vi "Obtain Request Events.vi"(8 "error in":errorcluster, 10 "Create New? (F)":bool) -> (0 "error out":errorcluster, 2 "testCoordinator Request Events":T1)   [LabVIEW 2026, in "testCoordinator.lvlib"]
doc: "This VI Obtains/Creates the Requests events that will be used for other modules to communicate with the module that owns this VI. These Requests events will be accessed only via Public API methods for this module.\n\n<b>NOTE</b>: The contents of this VI are automatically generated and modified by the <b>Tools > DQMH Consortium > DQMH</b> utilities. Consider using those utilities instead of making your own modifications to this VI.\n_____\nBased on DQMH Dev Tools: Project Template 7.1.2.1547."
uses:
  testCoordinator.lvlib
  Request Events--cluster.ctl
  Stop Argument--cluster.ctl
  Do Something Argument--cluster.ctl
  Do Something Else Argument--cluster.ctl
  Do Something Else and Wait for Reply Argument--cluster.ctl
  Do Something Else and Wait (Reply Payload)--cluster.ctl
  Show Panel Argument--cluster.ctl
  Hide Panel Argument--cluster.ctl
  Get Module Execution Status Argument--cluster.ctl
  Show Diagram Argument--cluster.ctl
  Set Manual Tests Folder Location Argument--cluster.ctl
  Set Manual Tests Folder Location (Reply Payload)--cluster.ctl
  Load Test Procedure Argument--cluster.ctl
  Begin Test Execution Argument--cluster.ctl
  Process Test Procedure Metadata Argument--cluster.ctl
  Instruction Completed Argument--cluster.ctl
  Process First Instruction Argument--cluster.ctl
  Load Next Test Case Argument--cluster.ctl
  Execute Launcher Argument--cluster.ctl
panel:
  # "NOTE: The contents of this VI are automatically generated and modified by the Tools > DQMH Consortium > DQMH utilities. Consider using those utilities instead of making your own modifications to this VI."
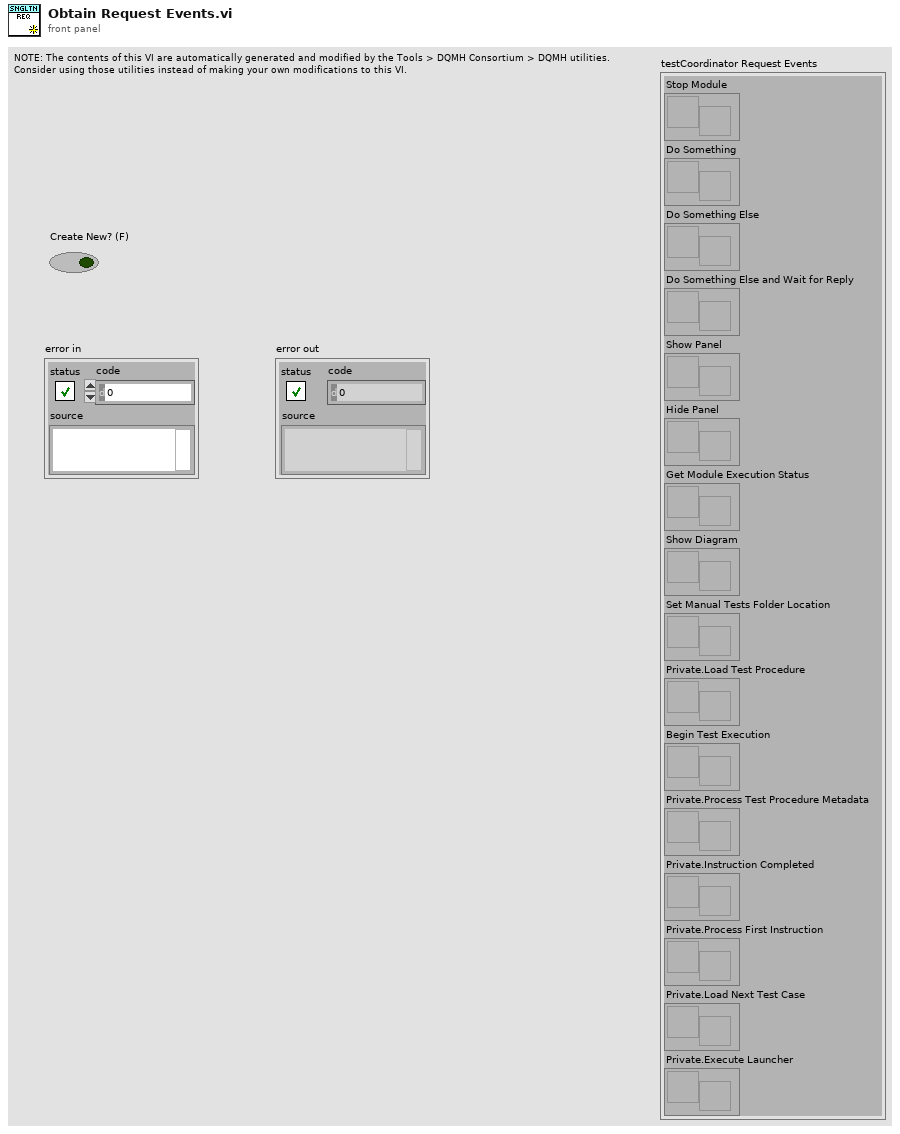
[diagram p1: front panel]
types:
  T1 = typedef "testCoordinator.lvlib/Request Events--cluster.ctl" = cluster{"Stop Module":refnum<user-event>, "Do Something":refnum<user-event>, "Do Something Else":refnum<user-event>, "Do Something Else and Wait for Reply":refnum<user-event>, "Show Panel":refnum<user-event>, "Hide Panel":refnum<user-event>, "Get Module Execution Status":refnum<user-event>, "Show Diagram":refnum<user-event>, "Set Manual Tests Folder Location":refnum<user-event>, "Private.Load Test Procedure":refnum<user-event>, "Begin Test Execution":refnum<user-event>, "Private.Process Test Procedure Metadata":refnum<user-event>, "Private.Instruction Completed":refnum<user-event>, "Private.Process First Instruction":refnum<user-event>, "Private.Load Next Test Case":refnum<user-event>, "Private.Execute Launcher":refnum<user-event>}
  T2 = typedef "testCoordinator.lvlib/Execute Launcher Argument--cluster.ctl" = cluster{"Boolean":bool}
  T3 = typedef "testCoordinator.lvlib/Load Next Test Case Argument--cluster.ctl" = cluster{"Boolean":bool}
  T4 = typedef "testCoordinator.lvlib/Process First Instruction Argument--cluster.ctl" = cluster{"Boolean":bool}
  T5 = typedef "testCoordinator.lvlib/Instruction Completed Argument--cluster.ctl" = cluster{"Boolean":bool}
  T6 = typedef "testCoordinator.lvlib/Process Test Procedure Metadata Argument--cluster.ctl" = cluster{"Boolean":bool}
  T7 = typedef "testCoordinator.lvlib/Begin Test Execution Argument--cluster.ctl" = cluster{"Test Procedure":string}
  T8 = typedef "testCoordinator.lvlib/Load Test Procedure Argument--cluster.ctl" = cluster{"Test Procedure File Name":string}
  T9 = typedef "testCoordinator.lvlib/Set Manual Tests Folder Location Argument--cluster.ctl" = cluster{"Manual Tests Folder":path, "Wait Notifier":refnum<notifier>, "wait for reply":bool}
  T10 = typedef "testCoordinator.lvlib/Hide Panel Argument--cluster.ctl" = cluster{"Hide Panel?":bool}
  T11 = typedef "testCoordinator.lvlib/Show Panel Argument--cluster.ctl" = cluster{"Show Panel?":bool}
  T12 = typedef "testCoordinator.lvlib/Show Diagram Argument--cluster.ctl" = cluster{"Debug?":bool}
  T13 = typedef "testCoordinator.lvlib/Get Module Execution Status Argument--cluster.ctl" = cluster{"Running?":bool}
  T14 = typedef "testCoordinator.lvlib/Do Something Else and Wait for Reply Argument--cluster.ctl" = cluster{"Do Something Else Msg":string, "X":dbl, "Wait Notifier":refnum<notifier>, "wait for reply":bool}
  T15 = typedef "testCoordinator.lvlib/Do Something Else Argument--cluster.ctl" = cluster{"Do Something Else Msg":string, "X":dbl}
  T16 = typedef "testCoordinator.lvlib/Do Something Argument--cluster.ctl" = cluster{"Do Something Msg":string}
  T17 = typedef "testCoordinator.lvlib/Stop Argument--cluster.ctl" = cluster{"Origin":string, "Exit via Stop Module Req?":bool, "Wait for Module to stop?":bool}
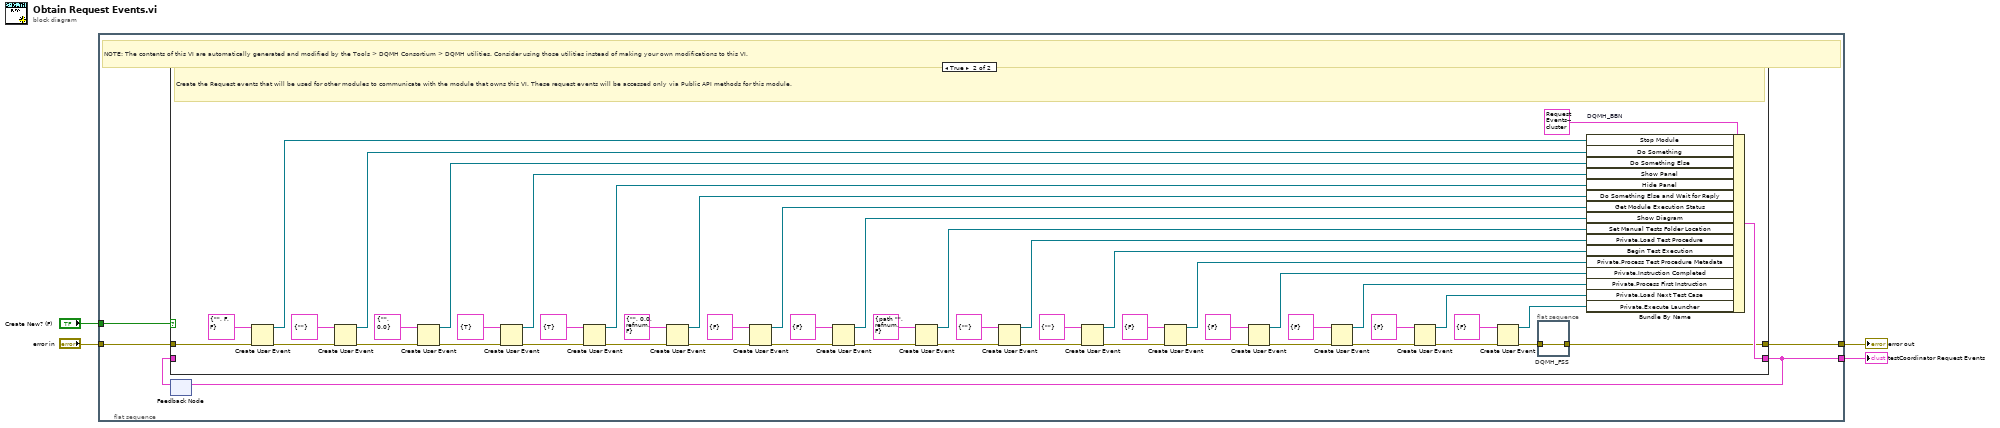
[diagram p0: block diagram]
diagram:
  n1 = flat-sequence {
    tunnel: [w9] -> w4
    tunnel: "error in" -> [w8]
    tunnel: [w6] -> w2
    tunnel: "Create New? (F)" -> [w5]
    frame #0 {
      # "NOTE: The contents of this VI are automatically generated and modified by the Tools > DQMH Consortium > DQMH utilities. Consider using those utilities instead of making your own modifications to this VI."
      n2 = feedback #1() -> (w7:T1)  [unwired: 1 in]
      n3 = case shown="True" w5 {
        tunnel: [w10 w44] -> w9
        tunnel: w8 -> [w10 w63]
        tunnel: [w11 w60] -> w6
        tunnel: w7 -> [w11 _]
        frame False {
          # "Obtain the Request events that were created in a previous call to this VI."
        }
        frame True {
          # "Create the Request events that will be used for other modules to communicate with the module that owns this VI. These request events will be accessed only via Public API methods for this module."
          n4 = Create User Event(user event datatype=T17 {"Origin"="", "Exit via Stop Module Req?"=FALSE, "Wait for Module to stop?"=FALSE} ("Stop Argument"), error in=w63) -> (user event=w61:refnum<user-event>, error out=w57:errorcluster)
          n5 = Create User Event(user event datatype=T16 {"Do Something Msg"=""} ("Do Something Argument"), error in=w57) -> (user event=w56:refnum<user-event>, error out=w55:errorcluster)
          n6 = Create User Event(user event datatype=T15 {"Do Something Else Msg"="", "X"=0.0} ("Do Something Else Argument"), error in=w55) -> (user event=w53:refnum<user-event>, error out=w52:errorcluster)
          n7 = Create User Event(user event datatype=T11 {"Show Panel?"=TRUE} ("Show Panel Argument"), error in=w52) -> (user event=w51:refnum<user-event>, error out=w50:errorcluster)
          n8 = Create User Event(user event datatype=T10 {"Hide Panel?"=TRUE} ("Hide Panel Argument"), error in=w50) -> (user event=w49:refnum<user-event>, error out=w48:errorcluster)
          n9 = Create User Event(user event datatype=T14 {"Do Something Else Msg"="", "X"=0.0, "Wait Notifier"=refnum, "wait for reply"=FALSE} ("Do Something Else and Wait for Reply Argument"), error in=w48) -> (user event=w47:refnum<user-event>, error out=w45:errorcluster)
          n10 = Create User Event(user event datatype=T13 {"Running?"=FALSE} ("Get Module Execution Status Argument"), error in=w45) -> (user event=w42:refnum<user-event>, error out=w43:errorcluster)
          n11 = Create User Event(user event datatype=T12 {"Debug?"=FALSE} ("Show Diagram Argument"), error in=w43) -> (user event=w39:refnum<user-event>, error out=w40:errorcluster)
          n12 = Create User Event(user event datatype=T9 {"Manual Tests Folder"=path "", "Wait Notifier"=refnum, "wait for reply"=FALSE} ("Set Manual Tests Folder Location Argument"), error in=w40) -> (user event=w34:refnum<user-event>, error out=w35:errorcluster)
          n13 = Create User Event(user event datatype=T8 {"Test Procedure File Name"=""} ("Load Test Procedure Argument"), error in=w35) -> (user event=w31:refnum<user-event>, error out=w32:errorcluster)
          n14 = Create User Event(user event datatype=T7 {"Test Procedure"=""} ("Begin Test Execution Argument"), error in=w32) -> (user event=w28:refnum<user-event>, error out=w29:errorcluster)
          n15 = Create User Event(user event datatype=T6 {"Boolean"=FALSE} ("Process Test Procedure Metadata Argument"), error in=w29) -> (user event=w25:refnum<user-event>, error out=w26:errorcluster)
          n16 = Create User Event(user event datatype=T5 {"Boolean"=FALSE} ("Instruction Completed Argument"), error in=w26) -> (user event=w22:refnum<user-event>, error out=w23:errorcluster)
          n17 = Create User Event(user event datatype=T4 {"Boolean"=FALSE} ("Process First Instruction Argument"), error in=w23) -> (user event=w19:refnum<user-event>, error out=w20:errorcluster)
          n18 = Create User Event(user event datatype=T3 {"Boolean"=FALSE} ("Load Next Test Case Argument"), error in=w20) -> (user event=w16:refnum<user-event>, error out=w17:errorcluster)
          n19 = Create User Event(user event datatype=T2 {"Boolean"=FALSE} ("Execute Launcher Argument"), error in=w17) -> (user event=w13:refnum<user-event>, error out=w14:errorcluster)
          n20 = flat-sequence "DQMH_FSS" {
            tunnel: w14 -> [w64]
            tunnel: [w64] -> w44
            frame #0 {
            }
          }
          n21 = Bundle By Name "DQMH_BBN"(cluster=T1 {"Stop Module"=refnum, "Do Something"=refnum, "Do Something Else"=refnum, "Do Something Else and Wait for Reply"=refnum, "Show Panel"=refnum, "Hide Panel"=refnum, "Get Module Execution Status"=refnum, "Show Diagram"=refnum, "Set Manual Tests Folder Location"=refnum, "Private.Load Test Procedure"=refnum, "Begin Test Execution"=refnum, "Private.Process Test Procedure Metadata"=refnum, "Private.Instruction Completed"=refnum, "Private.Process First Instruction"=refnum, "Private.Load Next Test Case"=refnum, "Private.Execute Launcher"=refnum} ("output cluster"), "Stop Module"=w61, "Do Something"=w56, "Do Something Else"=w53, "Show Panel"=w51, "Hide Panel"=w49, "Do Something Else and Wait for Reply"=w47, "Get Module Execution Status"=w42, "Show Diagram"=w39, "Set Manual Tests Folder Location"=w34, "Private.Load Test Procedure"=w31, "Begin Test Execution"=w28, "Private.Process Test Procedure Metadata"=w25, "Private.Instruction Completed"=w22, "Private.Process First Instruction"=w19, "Private.Load Next Test Case"=w16, "Private.Execute Launcher"=w13) -> (w60:T1)
        }
      }
      n22 = feedback-in #1(w6) -> ()
    }
  }
  "testCoordinator Request Events" <- w2
  "error out" <- w4
